vi "Close.vi"(8 "error in (no error)":errorcluster, 11 "UserEventActivationHandler in":refnum<class "UserEventActivationHandler.lvclass">) -> (0 "error out":errorcluster)   [LabVIEW 2026, in "ToastNotification.lvlib" / "UserEventActivationHandler.lvclass"]
doc: "Destroy the User Event stored in this handler and merge any cleanup error with the incoming error. Called by ToastService.Close. The caller must first unregister its receiving event registration. Cleanup is attempted even on incoming error. This method does not clear the stored reference or provide callback-drain or repeated-close guarantees; lifetime hardening remains tracked separately."
uses:
  UserEventActivationHandler.lvclass
  UserEventActivationHandler.lvclass/UserEventActivationHandler.ctl
  Read Event Ref.vi
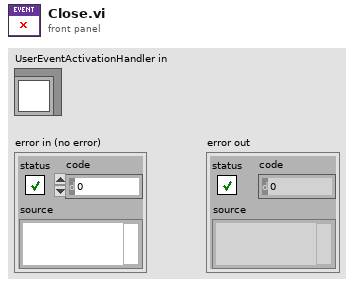
[diagram p1: front panel]
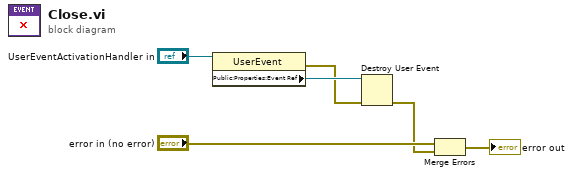
[diagram p0: block diagram]
diagram:
  n1 = property class="UserEvent"(reference="UserEventActivationHandler in") -> (error out=w2:errorcluster, "Public:Properties:Event Ref"=w3:refnum<user-event>)  [unwired: 1 in, 1 out]
  n2 = Destroy User Event(user event=w3, error in=w2) -> (error out=w1:errorcluster)
  n3 = Merge Errors("error in (no error)", w1) -> (→"error out":errorcluster)
